vi "Power Reset.vi"() -> (0 "error out":errorcluster, 2 "Result":string, 3 "Result":bool)   [LabVIEW 2021]
uses:
  10054_Control Folder/Support/Relay_no.ctl
panel:
  out "status":bool
  in  "error in (no error)":errorcluster
  out ".not. x?":bool
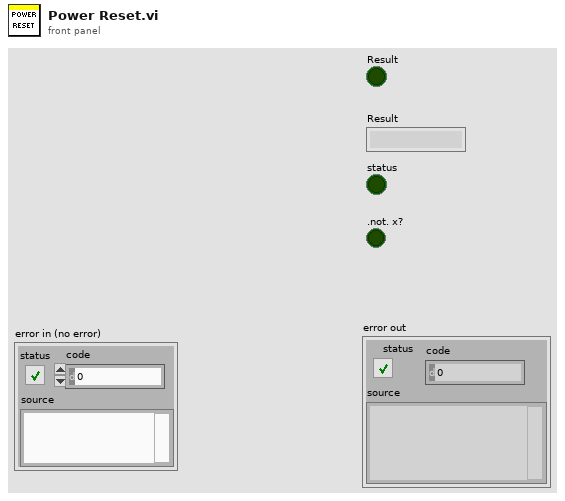
[diagram p1: front panel]
types:
  T1 = typedef "Relay_no.ctl" = enum16{"Init", "write&Read", "PCB Serial Write & Read", "PCB Write SSD & Password", "Read Wifi state", "Reset", "Close"}
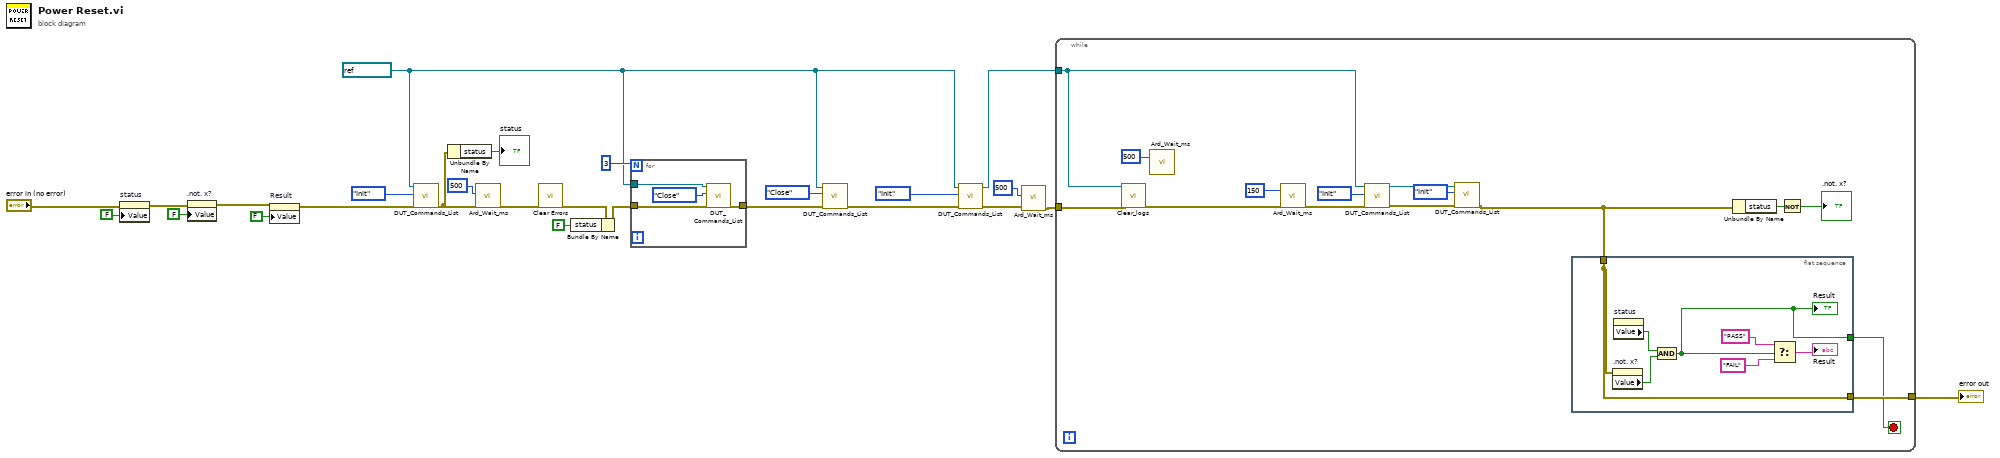
[diagram p0: block diagram]
diagram:
  w8 = refnum<visa-resource-name> "COM3" ("Resource In")
  n1 = property on="status" class="Bool (strict)"(error in="error in (no error)", "Value"=FALSE ("status")) -> (error out=w7:errorcluster)  [unwired: 1 in, 1 out]
  n2 = property on=".not. x?" class="Bool (strict)"(error in=w7, "Value"=FALSE (".not. x?")) -> (error out=w6:errorcluster)  [unwired: 1 in, 1 out]
  n3 = property on="Result" class="Bool (strict)"(error in=w6, "Value"=FALSE ("Result")) -> (error out=w5:errorcluster)  [unwired: 1 in, 1 out]
  n4 = call "DUT_Commands_List.vi"("error in"=w5, "Operation"=Relay_no."Init", "Resource In"=w8) -> ("error out"=w22:errorcluster)  [unwired: 6 in, 2 out]
  n5 = Unbundle By Name(w22) -> ("status"=→"status":bool)
  n6 = call "Ard_Wait_ms.vi"("error in"=w22, "millisec"=u32 500) -> ("error in 2"=w21:errorcluster)  [unwired: 9 in]
  n7 = call <vilib>:"Clear Errors.vi"("error in (no error)"=w21) -> ("error out"=w19:errorcluster)  [unwired: 5 in, 1 out]
  n8 = Bundle By Name(cluster=w19, "status"=FALSE) -> (w17:errorcluster)
  n9 = for {
    N: 3 -> [_]
    tunnel: w8 -> [w27]
    tunnel: w17 -> [w29]
    tunnel: [w28] -> w15
    n10 = call "DUT_Commands_List.vi"("error in"=w29, "Operation"=Relay_no."Close", "Resource In"=w27) -> ("error out"=w28:errorcluster)  [unwired: 6 in, 2 out]
  }
  n11 = call "DUT_Commands_List.vi"("error in"=w15, "Operation"=Relay_no."Close", "Resource In"=w8) -> ("error out"=w14:errorcluster)  [unwired: 6 in, 2 out]
  n12 = call "DUT_Commands_List.vi"("error in"=w14, "Operation"=Relay_no."Init", "Resource In"=w8) -> ("error out"=w10:errorcluster, "Resource out"=w1:refnum<visa-resource-name>)  [unwired: 6 in, 1 out]
  n13 = call "Ard_Wait_ms.vi"("error in"=w10, "millisec"=u32 500) -> ("error in 2"=w9:errorcluster)  [unwired: 9 in]
  n14 = while {
    tunnel: [w39] -> w26
    tunnel: w9 -> [w36]
    tunnel: w1 -> [w37]
    stop <- w38 stop-if-true
    n15 = call "Clear_logs.vi"("error in (no error)"=w36, "VISA resource name"=w37) -> ("error out"=w43:errorcluster)  [unwired: 4 in, 3 out]
    n16 = call "Ard_Wait_ms.vi"("millisec"=u32 500) -> ()  [unwired: 10 in, 1 out]
    n17 = call "Ard_Wait_ms.vi"("error in"=w43, "millisec"=u32 150) -> ("error in 2"=w44:errorcluster)  [unwired: 9 in]
    n18 = call "DUT_Commands_List.vi"("error in"=w44, "Operation"=Relay_no."Init", "Resource In"=w37) -> ("error out"=w33:errorcluster, "Resource out"=w32:refnum<visa-resource-name>)  [unwired: 6 in, 1 out]
    n19 = call "DUT_Commands_List.vi"("error in"=w33, "Operation"=Relay_no."Init", "Resource In"=w32) -> ("error out"=w34:errorcluster)  [unwired: 6 in, 2 out]
    n20 = flat-sequence {
      tunnel: w34 -> [w48]
      tunnel: [w48] -> w39
      tunnel: [w47] -> w38
      frame #0 {
        n21 = property on=".not. x?" class="Bool (strict)"(error in=w48) -> ("Value"=w52:bool)  [unwired: 1 in, 2 out]
        n22 = property on="status" class="Bool (strict)"() -> ("Value"=w46:bool)  [unwired: 2 in, 2 out]
        n23 = And(x=w46, y=w52) -> (x .and. y?=w47:bool)
        "Result" <- w47
        n24 = Select(t="PASS", s=w47, f="FAIL") -> (s? t:f=→"Result":string)
      }
    }
    n25 = Unbundle By Name(w34) -> ("status"=w41:bool)
    n26 = Not(x=w41) -> (.not. x?=→".not. x?":bool)
  }
  "error out" <- w26
